vi "Get Serial Number.vi"(8 "error in (no error)":errorcluster, 9 "para2":u32, 10 "para1":string, 11 "para0":u32) -> (0 "error out":errorcluster, 2 "para1 out":string, 3 "function return":u32)   [LabVIEW 2011, in "HID_ARZ.lvlib"]
doc: "GET_SERIAL_NUMBER GetSerialNumber;"
uses:
  HID_ARZ.lvlib
  <userlib>/HID_ARZ/mcHID.dll
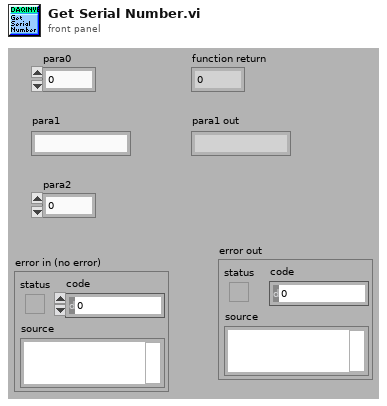
[diagram p1: front panel]
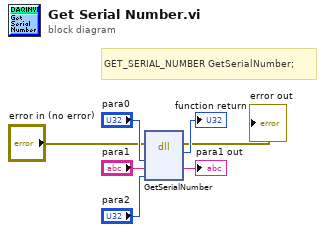
[diagram p0: block diagram]
diagram:
  # "GET_SERIAL_NUMBER GetSerialNumber;"
  n1 = dll-call lib="C:/Program Files (x86)/National Instruments/LabVIEW 2017/user.lib/HID_ARZ/mcHID.*" fn="GetSerialNumber"(error in="error in (no error)", "para0"="para0", "para1"="para1", "para2"="para2") -> (error out=→"error out":errorcluster, "return type"=→"function return":u32, "para1"=→"para1 out":string)  [unwired: 4 in, 1 out]
